vi "PicoScope6000ExampleAWG.vi"() -> ()   [LabVIEW 2010]
uses:
  ps6000.dll
panel:
  in  "General AWG Settings":T1={"Peak-to-Peak Voltage (microvolts)"=2000000, "Offset Voltage (microvolts)"=0, "Wave Type"=0, "Sweep Type"=0, "Shots"=0, "Sweeps"=0, "Trigger Type"=0, "Trigger Source"=0, "Ext. Threshold (ADC count)"=0, "White Noise/PRBS"=0} {"White Noise/PRBS" items=["Normal", "White Noise", "PRBS"]; "Trigger Source" items=["None", "Scope Trigger", "Aux. In", "Ext. In", "Software Trigger"]; "Trigger Type" items=["Rising", "Falling", "Gate High", "Gate Low"]; "Sweep Type" items=["Up", "Down", "Up-Down", "Down-Up"]; "Wave Type" items=["Sine", "Square", "Triangle", "Ramp Up", "Ramp Down", "Sinc", "Gaussian", "Half Sine", "DC", "Arbitrary"]}
  in  "error in (no error)":errorcluster
  out "Device Info":T2
  in  "Serial Number":string
  in  "Use Serial Number":bool
  in  "Arbitrary Waveform Settings":T3={"Arbirary waveform file path"=path "", "Start Delta Phase"=1000, "Index Mode"=0, "Stop Delta Phase"=1000, "Delta Phase Increment"=0, "Dwell Count"=0} {"Index Mode" items=["Single", "Dual", "Quad"]}
  in  "Stop S/W \nTrigger":bool
  in  "Apply Settings":bool
  in  "Stop VI":bool
  in  "Software \nTrigger":bool
  out "Arbitrary\nWaveform Graph":i16[](graph)
  in  "Standard Waveform Settings":T4={"Start Frequency (Hz)"=1000.0, "Stop Frequency (Hz)"=1000.0, "Increment (Hz)"=0.0, "Dwell Time (seconds)"=0.0} {"Start Frequency (Hz)" min=1 max=1000000}
  # "If Software trigger is selected, press the 'Stop S/W Trigger'\nbutton prior to selecting 'Apply Settings' or 'Stop VI'."
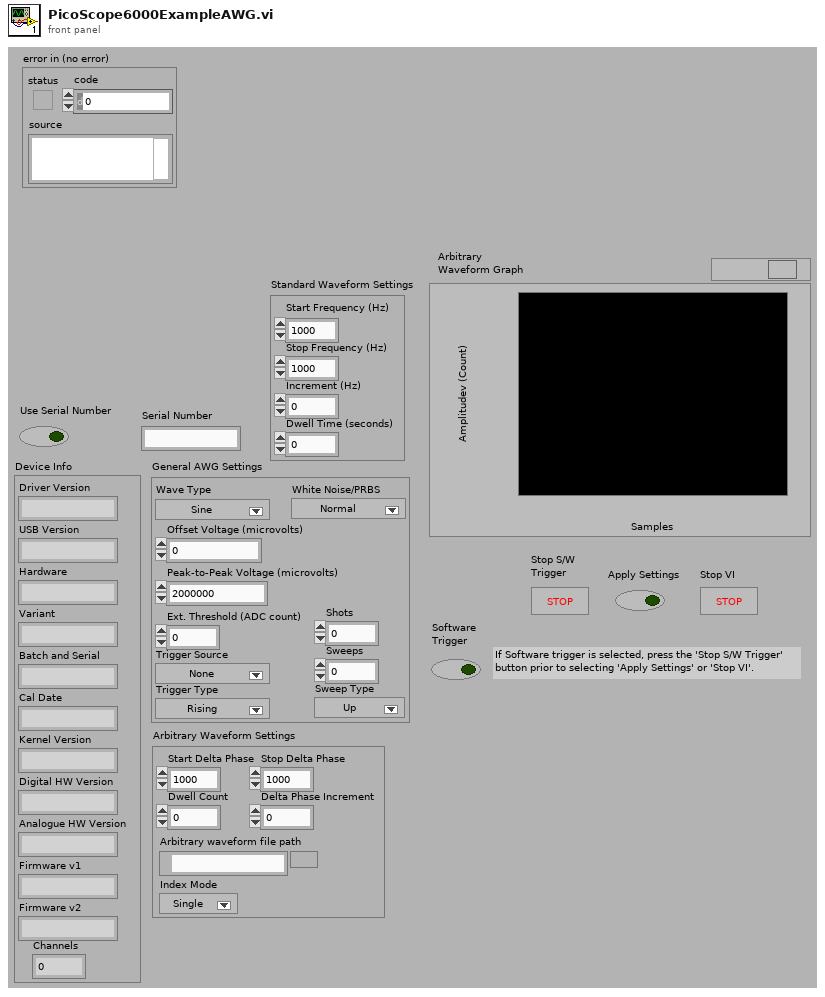
[diagram p1: front panel]
types:
  T1 = cluster{"Peak-to-Peak Voltage (microvolts)":u32, "Offset Voltage (microvolts)":i32, "Wave Type":u32, "Sweep Type":u32, "Shots":u32, "Sweeps":u32, "Trigger Type":u32, "Trigger Source":u32, "Ext. Threshold (ADC count)":i16, "White Noise/PRBS":u32}
  T2 = cluster{"Driver Version":string, "USB Version":string, "Hardware":string, "Variant":string, "Batch and Serial":string, "Cal Date":string, "Kernel Version":string, "Digital HW Version":string, "Analogue HW Version":string, "Firmware v1":string, "Firmware v2":string, "Channels":i16}
  T3 = cluster{"Arbirary waveform file path":path, "Start Delta Phase":u32, "Index Mode":i32, "Stop Delta Phase":u32, "Delta Phase Increment":u32, "Dwell Count":u32}
  T4 = cluster{"Start Frequency (Hz)":sgl, "Stop Frequency (Hz)":sgl, "Increment (Hz)":sgl, "Dwell Time (seconds)":sgl}
  T5 = cluster{"status":bool, "code":u32, "source":string}
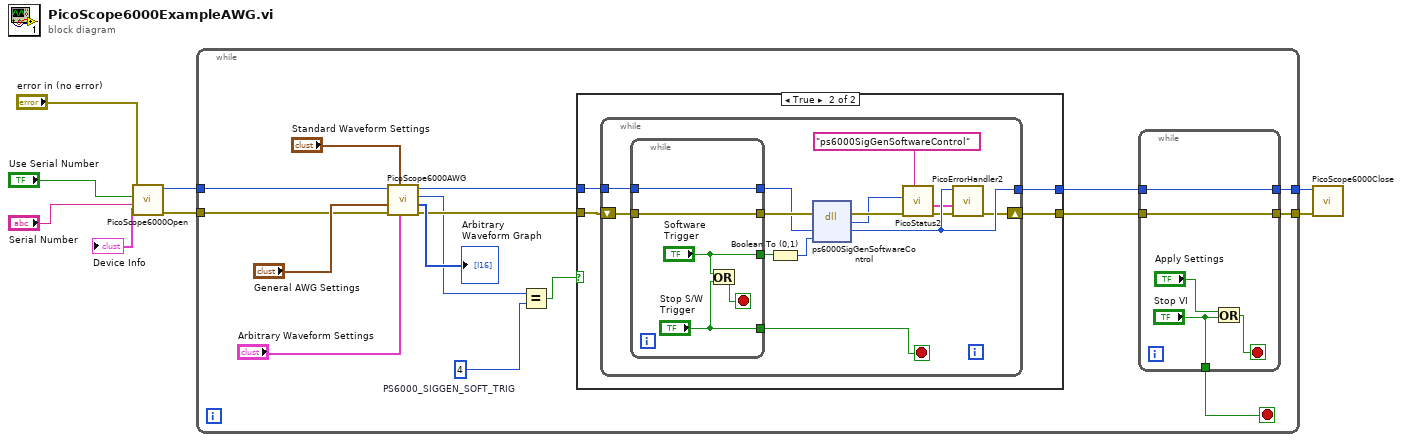
[diagram p0: block diagram]
diagram:
  n1 = call "PicoScope6000Open.vi"("error in (no error)"="error in (no error)", "Serial Number"="Serial Number", "Use Serial Number"="Use Serial Number") -> ("error out"=w7:errorcluster, "handle"=w8:i16, "Device Info"=→"Device Info":T2)  [unwired: 4 in, 2 out]
  n2 = while {
    tunnel: w8 -> [w12]
    tunnel: w7 -> [w13]
    tunnel: [w20] -> w6
    tunnel: [w14] -> w1
    stop <- w19 stop-if-true
    w22 = 4  # PS6000_SIGGEN_SOFT_TRIG
    n3 = call "PicoScope6000AWG.vi"("Arbitrary Waveform Settings"="Arbitrary Waveform Settings", "Standard Waveform Settings"="Standard Waveform Settings", "error in"=w13, "General AWG Settings"="General AWG Settings", "Handle In"=w12) -> ("error out"=w11:errorcluster, "Arbitrary\nWaveform Graph"=→"Arbitrary\nWaveform Graph":i16[], "Trigger Source Out"=w10:u32, "Handle Out"=w9:i16)  [unwired: 3 in]
    n4 = Equal?(x=w10, y=w22) -> (x = y?=w21:bool)
    n5 = case shown="True" w21 {
      tunnel: w11 -> [w30 w35]
      tunnel: [w31 w33] -> w17
      tunnel: w9 -> [w31 w34]
      tunnel: [w30 w32] -> w15
      frame False {
      }
      frame True {
        n6 = while {
          tunnel: w34 -> [w47]
          tunnel: [w45] -> w33
          shift-right: [w36] -> w32
          shift-left: w35 -> [w48]
          stop <- w41 stop-if-true
          n7 = while {
            tunnel: [w54] -> w49
            tunnel: w48 -> [w54]
            tunnel: ["Software \nTrigger"] -> w44
            tunnel: w47 -> [w53]
            tunnel: [w53] -> w46
            tunnel: ["Stop S/W \nTrigger"] -> w41
            stop <- w50 stop-if-true
            n8 = Or(x="Software \nTrigger", y="Stop S/W \nTrigger") -> (x .or. y?=w50:bool)
          }
          n9 = Boolean To (0,1)(Boolean=w44) -> (0, 1=w43:i16)
          n10 = dll-call lib="ps6000.dll" fn="ps6000SigGenSoftwareControl"(error in=w49, "handle"=w46, "state"=w43) -> (error out=w42:errorcluster, "PICO_STATUS"=w39:u32, "handle"=w45:i16)  [unwired: 3 in, 1 out]
          n11 = call "PicoStatus2.vi"("PICO source"="ps6000SigGenSoftwareControl" ("source"), "Error in"=w42, "PICO STATUS"=w39) -> ("error out"=w38:errorcluster, "PICO_STATUS out"=w37:T5)  [unwired: 5 in]
          n12 = call "PicoErrorHandler2.vi"("error in (no error)"=w38, "PICO_STATUS in"=w37, "handle In"=w45) -> ("error out"=w36:errorcluster)  [unwired: 8 in]
        }
      }
    }
    n13 = while {
      tunnel: ["Stop VI"] -> w19
      tunnel: [w29] -> w20
      tunnel: w17 -> [w29]
      tunnel: w15 -> [w25]
      tunnel: [w25] -> w14
      stop <- w28 stop-if-true
      n14 = Or(x="Apply Settings", y="Stop VI") -> (x .or. y?=w28:bool)
    }
  }
  n15 = call "PicoScope6000Close.vi"("error in (no error)"=w1, "handle"=w6) -> ()  [unwired: 8 in, 2 out]
